vi "VariantToCluster.vi"(8 "error in (no error)":errorcluster, 11 "Cluster":variant) -> (0 "error out":errorcluster, 2 "cluster elements info":variant[](array[variant]), 3 "Cluster elements":variant[](array[variant]))   [LabVIEW 2020, in "BlueVariantView.lvlib"]
uses:
  BlueVariantView.lvlib
  <vilib>/Utility/Data Type/NI_Data Type.lvlib
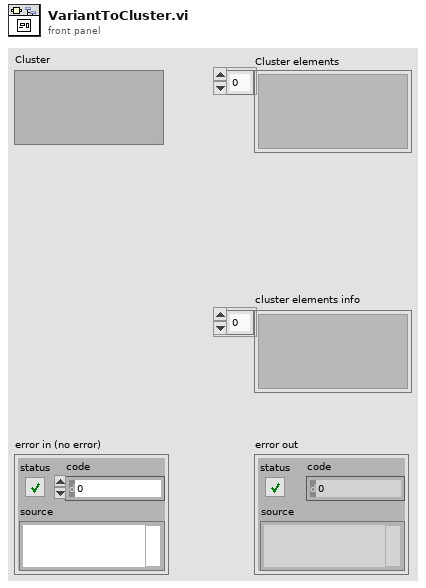
[diagram p1: front panel]
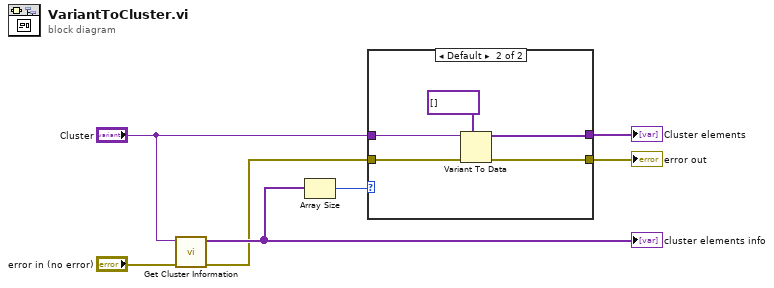
[diagram p0: block diagram]
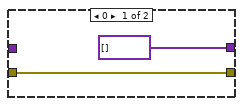
[diagram p2: hidden frame]
diagram:
  n1 = call <vilib>:"Get Cluster Information.vi"("error in (no error)"="error in (no error)", "variant"="Cluster") -> ("error out"=w2:errorcluster, "cluster elements"=w3:variant[])  [unwired: 8 in]
  "cluster elements info" <- w3
  n2 = Array Size(array=w3) -> (size(s)=w5:i32)
  n3 = case shown="Default" w5 {
    tunnel: "Cluster" -> [_ w13]
    tunnel: w2 -> [w8 w12]
    tunnel: [variant[] [] w11] -> w4
    tunnel: [w8 w10] -> w1
    frame 0 {
    }
    frame Default {
      n4 = Variant To Data(error in=w12, type=variant[] [], Variant=w13) -> (data=w11:variant[], error out=w10:errorcluster)
    }
  }
  "error out" <- w1
  "Cluster elements" <- w4
